vi "test Multi FPGA Synchronization.vi"(8 "error in (no error)":errorcluster, 11 "TestCase in":refnum<class "Engine Simulation Multi FPGA System Tests.lvclass">) -> (0 "error out":errorcluster, 3 "TestCase out":refnum<class "Engine Simulation Multi FPGA System Tests.lvclass">)   [LabVIEW 2020, in "Engine Simulation Multi FPGA System Tests.lvclass"]
uses:
  Engine Simulation Multi FPGA System Tests.lvclass
  C:/Program Files (x86)/National Instruments/LabVIEW 2020/vi.lib/NI/VeriStand Custom Device Testing Tools/VeriStandTestCase/VeriStandTestCase.lvclass
  <vilib>/NI VeriStand/Execution/Workspace/NI VeriStand - Set Single Channel Value.vi
  <vilib>/NI VeriStand/Execution/Workspace/NI VeriStand - Get Multiple Channel Values.vi
  <vilib>/addons/_JKI Toolkits/VI Tester/TestCase.llb/TestCase.lvclass
  <vilib>/NI VeriStand/Execution/Workspace/NI_VS Workspace ExecutionAPI.lvlib
  C:/Program Files (x86)/National Instruments/LabVIEW 2020/vi.lib/addons/_JKI Toolkits/VI Tester/TestCase.llb/TestCase.lvclass
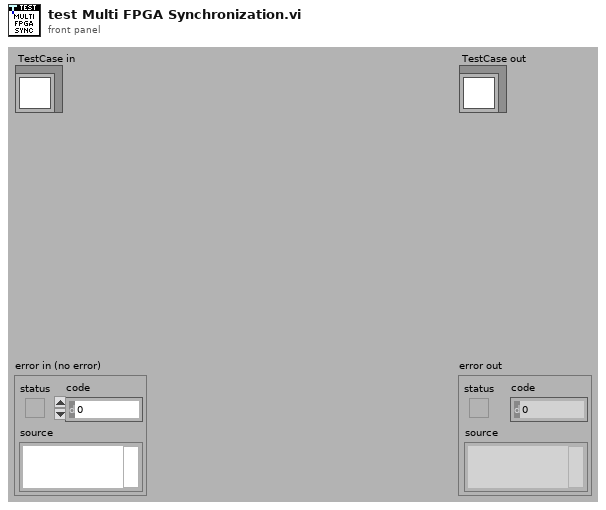
[diagram p1: front panel]
types:
  T1 = typedef "NI_VS Workspace ExecutionAPI.lvlib/WorkspaceAPI.ctl" = refnum<k24>
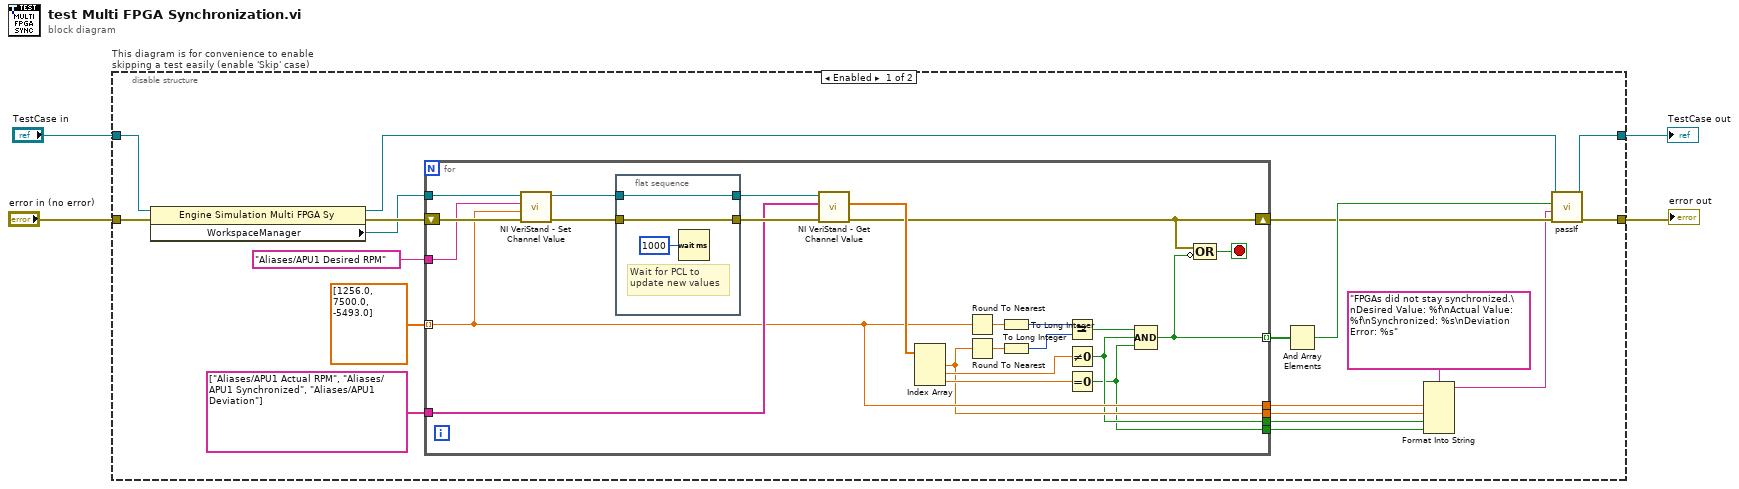
[diagram p0: block diagram]
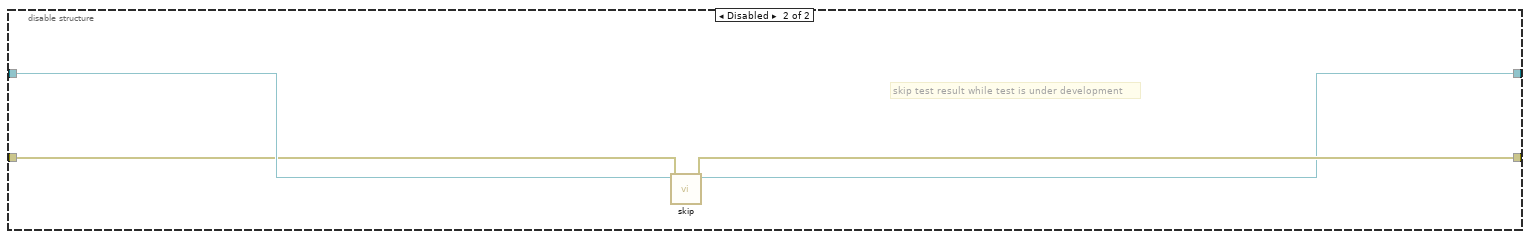
[diagram p2: hidden frame]
diagram:
  n1 = disable-structure "This diagram is for convenience to enable skipping a test easily (enable 'Skip' case)" shown="Enabled" {
    disable-tunnel: "TestCase in" -> [w23 w53]
    disable-tunnel: [w18 w51] -> w1
    disable-tunnel: [w17 w52] -> w3
    disable-tunnel: "error in (no error)" -> [w22 w50]
    frame Enabled {
      n2 = property class="Engine Simulation Multi FPGA Sy"(reference=w23, error in=w22) -> (reference out=w19:refnum<class "Engine Simulation Multi FPGA System Tests.lvclass">, error out=w21:errorcluster, "WorkspaceManager"=w20:T1)
      n3 = for {
        tunnel: "Aliases/APU1 Desired RPM" -> [w44]
        shift-right: [w29] -> w11
        shift-left: w21 -> [w46]
        tunnel: dbl[] [1256.0, 7500.0, -5493.0] -> [w27] mode=indexing
        tunnel: string[] ["Aliases/APU1 Actual RPM", "Aliases/APU1 Synchronized", "Aliases/APU1 Deviation"] -> [w32]
        tunnel: w20 -> [w45]
        tunnel: [w30] -> w13 mode=indexing
        tunnel: [w27] -> w9
        tunnel: [w26] -> w8
        tunnel: [w25] -> w7
        tunnel: [w24] -> w6
        stop <- w28 stop-if-true
        n4 = call-poly <vilib>:"NI VeriStand - Set Channel Value.vi"("error in (no error)"=w46, "Value"=w27, "Channel"=w44, "WorkspaceManager in"=w45) -> ("error out"=w34:errorcluster, "WorkspaceManager out"=w33:T1)  [unwired: 6 in]
        n5 = flat-sequence {
          tunnel: w33 -> [w48]
          tunnel: w34 -> [w49]
          tunnel: [w49] -> w37
          tunnel: [w48] -> w36
          frame #0 {
            # "Wait for PCL to\nupdate new values"
            n6 = Wait (ms)(milliseconds to wait=u32 1000) -> ()  [unwired: 1 out]
          }
        }
        n7 = call-poly <vilib>:"NI VeriStand - Get Channel Value.vi"("error in (no error)"=w37, "Channels"=w32, "WorkspaceManager in"=w36) -> ("error out"=w29:errorcluster, "Values"=w43:dbl[])  [unwired: 6 in, 1 out]
        n8 = Index Array(array=w43) -> (element #1=w26:dbl, element #2=w42:dbl, element #3=w41:dbl)  [unwired: 3 in]
        n9 = Round To Nearest(number=w27) -> (nearest integer value=w39:dbl)
        n10 = Round To Nearest(number=w26) -> (nearest integer value=w38:dbl)
        n11 = To Long Integer(number=w39) -> (32bit integer=w35:i32)
        n12 = To Long Integer(number=w38) -> (32bit integer=w31:i32)
        n13 = Equal?(x=w35, y=w31) -> (x = y?=w40:bool)
        n14 = Not Equal To 0?(x=w42) -> (x != 0?=w25:bool)
        n15 = Equal To 0?(x=w41) -> (x = 0?=w24:bool)
        n16 = Compound Arithmetic op=AND(w40, w25, w24) -> (w30:bool)
        n17 = Compound Arithmetic op=OR(w29, invert w30) -> (w28:bool)
      }
      n18 = And Array Elements(Boolean array=w13) -> (logical AND=w12:bool)
      n19 = Format Into String(format string="FPGAs did not stay synchronized.\nDesired Value: %f\nActual Value: %f\nSynchronized: %s\nDeviation Error: %s", w9, w8, w7, w6) -> (resulting string=w5:string)  [unwired: 2 in, 1 out]
      n20 = call-dynamic "passIf.vi"("error in (no error)"=w11, "message (\"\")"=w5, "pass"=w12, "TestCase in"=w19) -> ("error out"=w17:errorcluster, "TestCase out"=w18:refnum<class "Engine Simulation Multi FPGA System Tests.lvclass">)  [unwired: 6 in]
    }
    frame Disabled {
      # "skip test result while test is under development"
      n21 = call <vilib>:"skip.vi"("error in (no error)"=w50, "TestCase in"=w53) -> ("error out"=w52:errorcluster, "TestCase out"=w51:refnum<class "Engine Simulation Multi FPGA System Tests.lvclass">)  [unwired: 8 in]
    }
  }
  "error out" <- w3
  "TestCase out" <- w1
